vi "Evaluate.vi"(8 "error in (no error)":errorcluster, 11 "One In":refnum<class "One.lvclass">) -> (0 "error out":errorcluster, 1 "Message":string, 2 "Passed?":bool)   [LabVIEW 2020, in "One.lvlib" / "One.lvclass"]
uses:
  One.lvclass
  One.lvclass/One.ctl
  Core/VI Call/VI Call.lvclass
  Core/Comparator/Comparator.lvclass
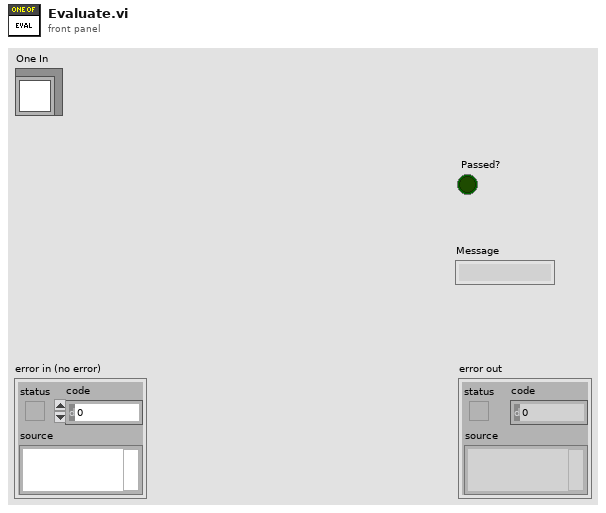
[diagram p1: front panel]
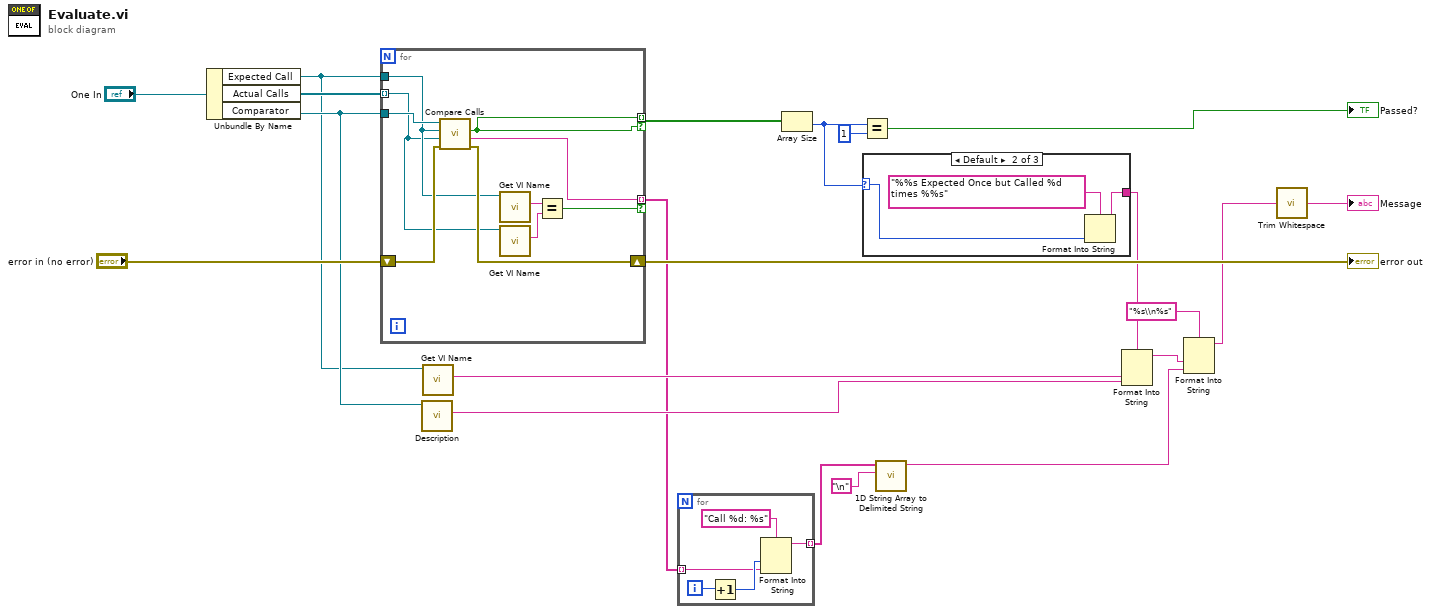
[diagram p0: block diagram]
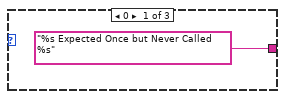
[diagram p2: hidden frame]
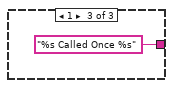
[diagram p3: hidden frame]
diagram:
  n1 = Unbundle By Name("One In") -> ("Expected Call"=w10:refnum<class "VI Call.lvclass">, "Actual Calls"=w19:refnum<class "VI Call.lvclass">[], "Comparator"=w15:refnum<class "Comparator.lvclass">)
  n2 = for {
    tunnel: w10 -> [w24]
    tunnel: w15 -> [w31]
    tunnel: w19 -> [w23] mode=indexing
    shift-right: [w29] -> w18
    shift-left: "error in (no error)" -> [w30]
    tunnel: [w28] -> w17 mode=indexing if=w28
    tunnel: [w27] -> w2 mode=indexing if=w22
    n3 = call-dynamic "Compare Calls.vi"("error in (no error)"=w30, "VI Call 2"=w23, "VI Call 1"=w24, "Comparator in"=w31) -> ("error out"=w29:errorcluster, "Description"=w27:string, "Equal?"=w28:bool)  [unwired: 5 in]
    n4 = call-dynamic "Get VI Name.vi"("VI Call In"=w24) -> ("VI Name"=w26:string)  [unwired: 9 in, 1 out]
    n5 = call-dynamic "Get VI Name.vi"("VI Call In"=w23) -> ("VI Name"=w25:string)  [unwired: 9 in, 1 out]
    n6 = Equal?(x=w26, y=w25) -> (x = y?=w22:bool)
  }
  "error out" <- w18
  n7 = call-dynamic "Description.vi"("Comparator in"=w15) -> ("Description"=w12:string)  [unwired: 9 in, 1 out]
  n8 = call-dynamic "Get VI Name.vi"("VI Call In"=w10) -> ("VI Name"=w9:string)  [unwired: 9 in, 1 out]
  n9 = for {
    tunnel: w2 -> [w33] mode=indexing
    tunnel: [w32] -> w1 mode=indexing
    i -> [w35]
    n10 = Increment(x=w35) -> (x+1=w34:i32)
    n11 = Format Into String(format string="Call %d: %s", w34, w33) -> (resulting string=w32:string)  [unwired: 2 in, 1 out]
  }
  n12 = Array Size(array=w17) -> (size(s)=w11:i32)
  n13 = Equal?(x=w11, y=1) -> (x = y?=→"Passed?":bool)
  n14 = case shown="Default" w11 {
    selector: w11 -> [_ w39 _]
    tunnel: ["%s Expected Once but Never Called %s" ("Message") w38 "%s Called Once %s" ("Message")] -> w14
    frame 0 {
    }
    frame Default {
      n15 = Format Into String(format string="%%s Expected Once but Called %d times %%s" ("Message"), w39) -> (resulting string=w38:string)  [unwired: 2 in, 1 out]
    }
    frame 1 {
    }
  }
  n16 = call <vilib>:"1D String Array to Delimited String.vi"("delimiter"="\n", "string array"=w1) -> ("delimited string"=w8:string)  [unwired: 9 in]
  n17 = Format Into String(format string=w14, w9, w12) -> (resulting string=w7:string)  [unwired: 2 in, 1 out]
  n18 = Format Into String(format string="%s\\n%s", w7, w8) -> (resulting string=w5:string)  [unwired: 2 in, 1 out]
  n19 = call <vilib>:"Trim Whitespace.vi"("string"=w5) -> ("trimmed string"=→"Message":string)  [unwired: 1 in]
